vi "stream waveform to channel.vi"(10 "Waveform":waveform(dbl), 11 "channel":refnum<class "Channel.lvclass">) -> (0 "error out":errorcluster)   [LabVIEW 2020, in "nominal core steps.lvlib"]
doc: "Streams a full waveform to the channel. Converts t0+dt to individual timestamps before sending."
uses:
  nominal core steps.lvlib
  <vilib>/Nominal/Nominal IO Client/submodules/nominal-streaming-labview-ffi/lv_src/Channel/Channel.lvclass
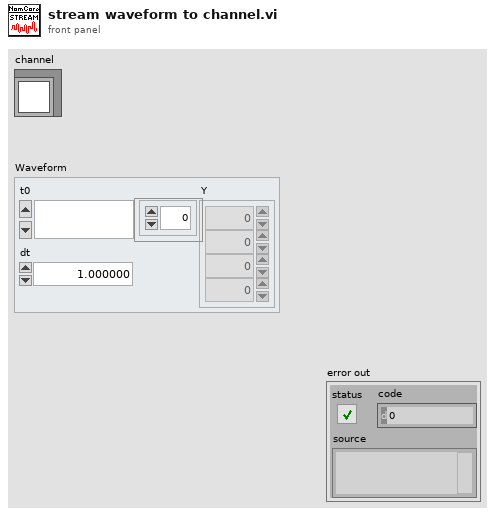
[diagram p1: front panel]
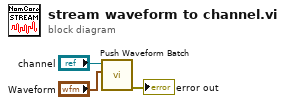
[diagram p0: block diagram]
diagram:
  n1 = call <vilib>:"Push Waveform Batch.vi"("Waveform"="Waveform", "Channel in"="channel") -> ("error out"=→"error out":errorcluster)  [unwired: 8 in, 1 out]
